vi "Completer tous seg.vi"(3 "Programme":cluster{"chaîne o":string, "Value":dbl}[][](array[cluster])) -> (1 "Programme avec tous les segments":cluster{"chaîne o":string, "Value":dbl}[][](array[cluster]))   [LabVIEW 2022 SP3]
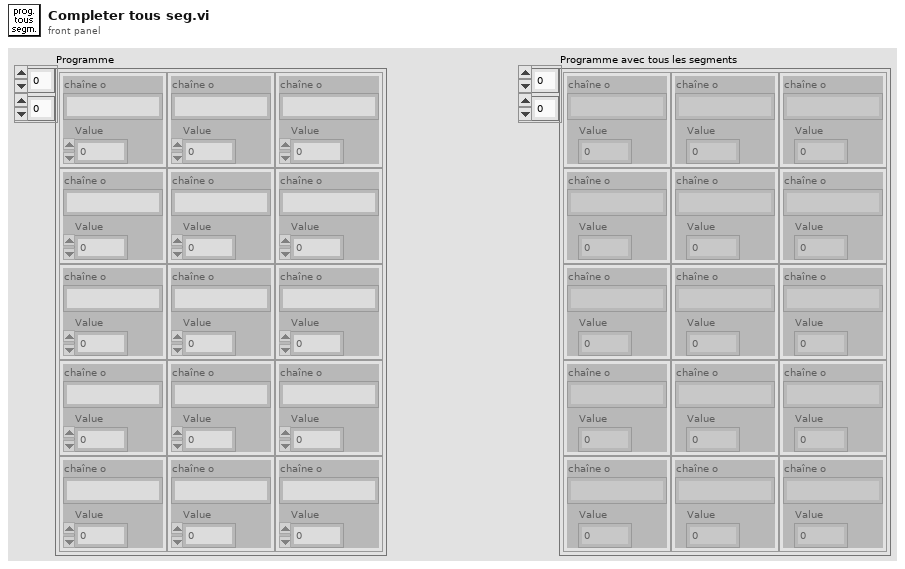
[diagram p1: front panel]
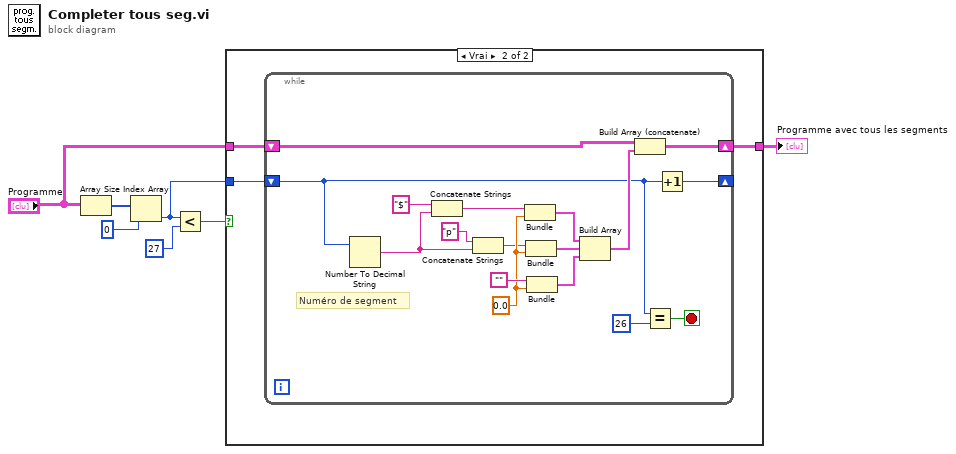
[diagram p0: block diagram]
diagram:
  n1 = Array Size(array="Programme") -> (size(s)=w7:i32[])
  n2 = Index Array(array=w7, index=0 ("indice")) -> (element=w2:i32)
  n3 = Less?(x=w2, y=27 ("cas vrai")) -> (x < y?=w5:bool)
  n4 = case shown="Vrai" w5 {
    tunnel: "Programme" -> [w8 w10]
    tunnel: [w8 w9] -> w3
    tunnel: w2 -> [_ w11]
    frame False {
    }
    frame True {
      n5 = while {
        shift-right: [w28] -> _
        shift-left: w11 -> [w14]
        shift-right: [w25] -> w9
        shift-left: w10 -> [w26]
        stop <- w27 stop-if-true
        w23 = 0.0
        # "Numéro de segment"
        n6 = Number To Decimal String(number=w14) -> (decimal integer string=w13:string)  [unwired: 1 in]
        n7 = Concatenate Strings("$", w13) -> (w17:string)
        n8 = Concatenate Strings("p", w13) -> (w15:string)
        n9 = Bundle(w17, w23) -> (w21:cluster{string, dbl})  [unwired: 1 in]
        n10 = Bundle(w15, w23) -> (w22:cluster{string, dbl})  [unwired: 1 in]
        n11 = Bundle("", w23) -> (w20:cluster{string, dbl})  [unwired: 1 in]
        n12 = Build Array(w21, w22, w20) -> (w19:cluster{string, dbl}[])
        n13 = Build Array (concatenate)(w26, w19) -> (w25:cluster{"chaîne o":string, "Value":dbl}[][])
        n14 = Equal?(x=w14, y=26 ("cas vrai")) -> (x = y?=w27:bool)
        n15 = Increment(x=w14) -> (x+1=w28:i32)
      }
    }
  }
  "Programme avec tous les segments" <- w3
